vi "KYFG Get Grabber Value String.vi"(0 "handle":u32, 5 "paramName":string, 7 "stringPtr":string, 9 "stringSize":u32, 11 "error in (no error)":errorcluster) -> (4 "handle out":u32(ring), 10 "stringValueOut":string, 15 "error out":errorcluster)   [LabVIEW 2023, in "KYFGLib_lv.lvlib"]
doc: "KYFG_API FGSTATUS KYFG_GetGrabberValueString(FGHANDLE handle, const char *paramName, char** ptr);"
uses:
  KYFGLib_lv.lvlib
  KYFGLib.dll
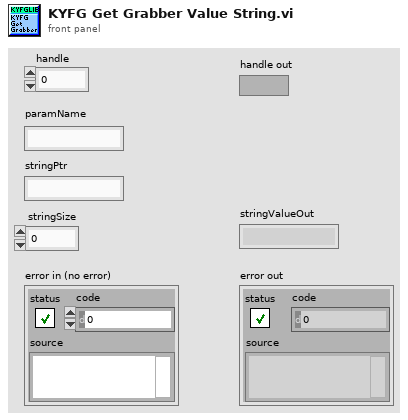
[diagram p1: front panel]
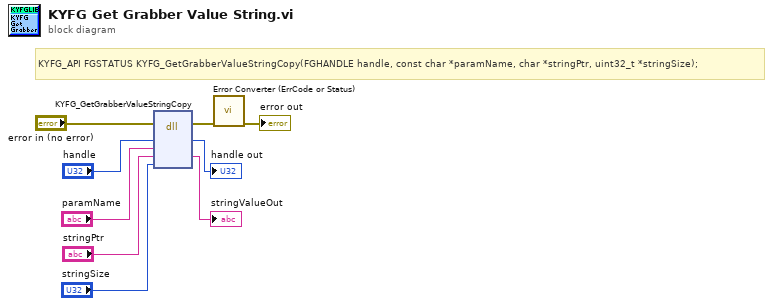
[diagram p0: block diagram]
diagram:
  # "KYFG_API FGSTATUS KYFG_GetGrabberValueStringCopy(FGHANDLE handle, const char *paramName, char *stringPtr, uint32_t *stringSize);"
  n1 = dll-call lib="KYFGLib.dll" fn="KYFG_GetGrabberValueStringCopy"(error in="error in (no error)", "handle"="handle", "paramName"="paramName", "stringPtr"="stringPtr", "stringSize"="stringSize") -> (error out=w5:errorcluster, "handle"=→"handle out":u32, "stringPtr"=→"stringValueOut":string)  [unwired: 5 in, 1 out]
  n2 = call "Error Converter (ErrCode or Status).vi"("error in (no error)"=w5) -> ("error out"=→"error out":errorcluster)  [unwired: 10 in]
